vi "Donnees fichier distant.vi"() -> (0 "Données":string[](array[string]), 1 "données présentes":bool)   [LabVIEW 2022 SP3]
uses:
  Variables globales/Variable glob Keller.vi
  Variables globales/Variable glob Leybold.vi
  Variables globales/Variable glob Edwards.vi
  Variables globales/Variable glob Th.vi
  Variables globales/Variable glob Pt.vi
  Variables globales/Variables glob EUROTHERM.vi
  Variables globales/Variable globale compteurs.vi
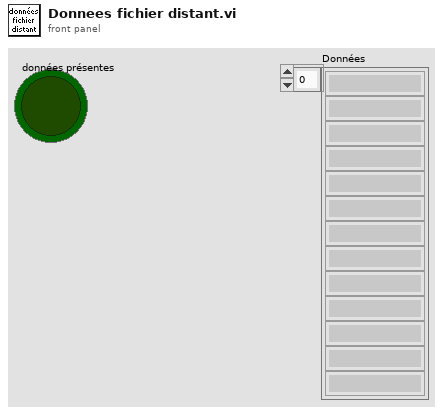
[diagram p1: front panel]
types:
  T1 = cluster{"Nom tache Pt":refnum<k21>, "Noms des Pt":string[], "Nb Pt":i16, "Selection Pt":bool[], "Nom Pt selectionnees":string[]}[]
  T2 = cluster{"Nom tache Th":refnum<k21>, "Noms des Th":string[], "Nb Th":i16, "Selection Th":bool[], "Nom Th selectionnes":string[]}[]
  T3 = cluster{"Nom tache compteurs":refnum<k21>, "Noms des compteurs":string[], "Selection":bool[], "Init compteurs":dbl[], "Noms compteurs selectionnes":string[]}
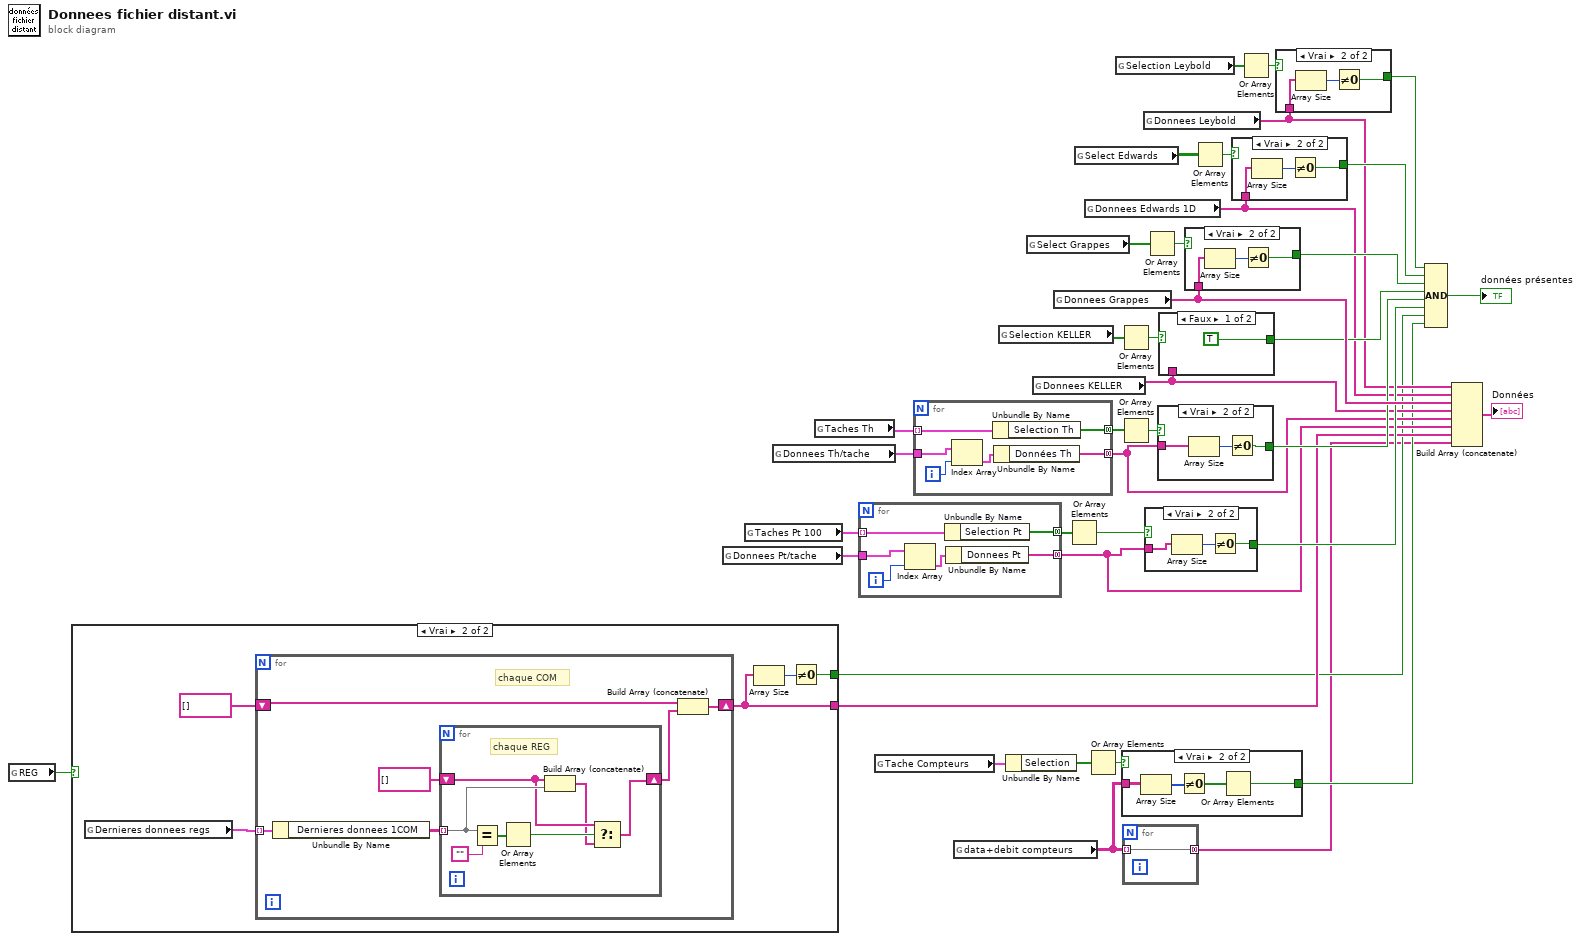
[diagram p0: block diagram]
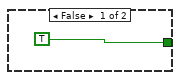
[diagram p2: hidden frame]
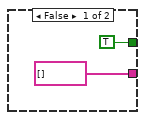
[diagram p3: hidden frame]
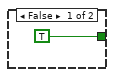
[diagram p4: hidden frame]
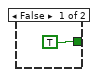
[diagram p5: hidden frame]
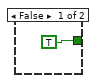
[diagram p6: hidden frame]
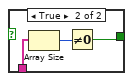
[diagram p7: hidden frame]
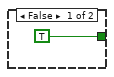
[diagram p8: hidden frame]
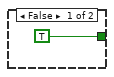
[diagram p9: hidden frame]
diagram:
  n1 = global read "Variables glob EUROTHERM.vi" "REG"() -> (w9:bool)
  n2 = case shown="Vrai" w9 {
    tunnel: [string[] [] w43] -> w8
    tunnel: [TRUE w42] -> w7
    frame False {
    }
    frame True {
      n3 = global read "Variables glob EUROTHERM.vi" "Dernieres donnees regs"() -> (w45:cluster{"Dernieres donnees 1COM":string[][]}[])
      n4 = for {
        tunnel: w45 -> [w48] mode=indexing
        shift-right: [w49] -> w43
        shift-left: string[] [] -> [w50]
        # "chaque COM"
        n5 = Unbundle By Name(w48) -> ("Dernieres donnees 1COM"=w47:string[][])
        n6 = for {
          tunnel: w47 -> [w59] mode=indexing
          shift-right: [w53] -> w51
          shift-left: string[] [] -> [w55]
          # "chaque REG"
          n7 = Equal?(x=w59, y="") -> (x = y?=w57:bool[])
          n8 = Or Array Elements(Boolean array=w57) -> (logical OR=w56:bool)
          n9 = Build Array (concatenate)(w55, w59) -> (w54:string[])
          n10 = Select(t=w55, s=w56, f=w54) -> (s? t:f=w53:string[])
        }
        n11 = Build Array (concatenate)(w50, w51) -> (w49:string[])
      }
      n12 = Array Size(array=w43) -> (size(s)=w44:i32)
      n13 = Not Equal To 0?(x=w44) -> (x != 0?=w42:bool)
    }
  }
  n14 = global read "Variable glob Pt.vi" "Donnees Pt/tache"() -> (w11:cluster{"Donnees Pt":string[]}[])
  n15 = global read "Variable glob Pt.vi" "Taches Pt 100"() -> (w17:T1)
  n16 = global read "Variable glob Th.vi" "Donnees Th/tache"() -> (w10:cluster{"Données Th":string[]}[])
  n17 = global read "Variable glob Th.vi" "Taches Th"() -> (w14:T2)
  n18 = for {
    tunnel: w17 -> [w64] mode=indexing
    tunnel: [w65] -> w16 mode=concatenating
    tunnel: [w63] -> w12 mode=concatenating
    tunnel: w11 -> [w61]
    i -> [w62]
    n19 = Index Array(array=w61, index=w62) -> (element=w60:cluster{"Donnees Pt":string[]})
    n20 = Unbundle By Name(w64) -> ("Selection Pt"=w65:bool[])
    n21 = Unbundle By Name(w60) -> ("Donnees Pt"=w63:string[])
  }
  n22 = global read "Variable globale compteurs.vi" "Tache Compteurs"() -> (w4:T3)
  n23 = for {
    tunnel: w14 -> [w71] mode=indexing
    tunnel: [w70] -> w15 mode=concatenating
    tunnel: [w69] -> w13 mode=concatenating
    tunnel: w10 -> [w68]
    i -> [w67]
    n24 = Index Array(array=w68, index=w67) -> (element=w66:cluster{"Données Th":string[]})
    n25 = Unbundle By Name(w71) -> ("Selection Th"=w70:bool[])
    n26 = Unbundle By Name(w66) -> ("Données Th"=w69:string[])
  }
  n27 = global read "Variable globale compteurs.vi" "data+debit compteurs"() -> (w6:string[][])
  n28 = global read "Variable glob Keller.vi" "Selection KELLER"() -> (w21:bool[])
  n29 = Unbundle By Name(w4) -> ("Selection"=w5:bool[])
  n30 = global read "Variable glob Edwards.vi" "Select Grappes"() -> (w37:bool[])
  n31 = global read "Variable glob Keller.vi" "Donnees KELLER"() -> (w28:string[])
  n32 = global read "Variable glob Edwards.vi" "Donnees Grappes"() -> (w38:string[])
  n33 = Or Array Elements(Boolean array=w16) -> (logical OR=w32:bool)
  n34 = global read "Variable glob Edwards.vi" "Select Edwards"() -> (w20:bool[][])
  n35 = global read "Variable glob Edwards.vi" "Donnees Edwards 1D"() -> (w25:string[])
  n36 = Or Array Elements(Boolean array=w5) -> (logical OR=w3:bool)
  n37 = global read "Variable glob Leybold.vi" "Selection Leybold"() -> (w18:bool[])
  n38 = Or Array Elements(Boolean array=w21) -> (logical OR=w27:bool)
  n39 = Or Array Elements(Boolean array=w15) -> (logical OR=w30:bool)
  n40 = case shown="Vrai" w3 {
    tunnel: w6 -> [_ w76]
    tunnel: [TRUE w73] -> w2
    frame False {
    }
    frame True {
      n41 = Array Size(array=w76) -> (size(s)=w75:i32[])
      n42 = Not Equal To 0?(x=w75) -> (x != 0?=w74:bool[])
      n43 = Or Array Elements(Boolean array=w74) -> (logical OR=w73:bool)
    }
  }
  n44 = for {
    tunnel: w6 -> [w77] mode=indexing
    tunnel: [w77] -> w1 mode=concatenating
  }
  n45 = global read "Variable glob Leybold.vi" "Donnees Leybold"() -> (w19:string[])
  n46 = case shown="Vrai" w32 {
    tunnel: [TRUE w80] -> w33
    tunnel: w12 -> [_ w79]
    frame False {
    }
    frame True {
      n47 = Array Size(array=w79) -> (size(s)=w81:i32)
      n48 = Not Equal To 0?(x=w81) -> (x != 0?=w80:bool)
    }
  }
  n49 = Or Array Elements(Boolean array=w37) -> (logical OR=w36:bool)
  n50 = case shown="Vrai" w30 {
    tunnel: [TRUE w84] -> w31
    tunnel: w13 -> [_ w83]
    frame False {
    }
    frame True {
      n51 = Array Size(array=w83) -> (size(s)=w85:i32)
      n52 = Not Equal To 0?(x=w85) -> (x != 0?=w84:bool)
    }
  }
  n53 = case shown="Faux" w27 {
    tunnel: w28 -> [_ w89]
    tunnel: [TRUE w87] -> w29
    frame False {
    }
    frame True {
      n54 = Array Size(array=w89) -> (size(s)=w88:i32)
      n55 = Not Equal To 0?(x=w88) -> (x != 0?=w87:bool)
    }
  }
  n56 = case shown="Vrai" w36 {
    tunnel: w38 -> [_ w93]
    tunnel: [TRUE w91] -> w39
    frame False {
    }
    frame True {
      n57 = Array Size(array=w93) -> (size(s)=w92:i32)
      n58 = Not Equal To 0?(x=w92) -> (x != 0?=w91:bool)
    }
  }
  n59 = Or Array Elements(Boolean array=w20) -> (logical OR=w24:bool)
  n60 = case shown="Vrai" w24 {
    tunnel: w25 -> [_ w97]
    tunnel: [TRUE w95] -> w26
    frame False {
    }
    frame True {
      n61 = Array Size(array=w97) -> (size(s)=w96:i32)
      n62 = Not Equal To 0?(x=w96) -> (x != 0?=w95:bool)
    }
  }
  n63 = Or Array Elements(Boolean array=w18) -> (logical OR=w22:bool)
  n64 = case shown="Vrai" w22 {
    tunnel: w19 -> [_ w101]
    tunnel: [TRUE w99] -> w23
    frame False {
    }
    frame True {
      n65 = Array Size(array=w101) -> (size(s)=w100:i32)
      n66 = Not Equal To 0?(x=w100) -> (x != 0?=w99:bool)
    }
  }
  n67 = Compound Arithmetic op=AND(w23, w26, w39, w29, w31, w33, w7, w2) -> (→"données présentes":bool)
  n68 = Build Array (concatenate)(w19, w25, w38, w28, w13, w12, w8, w1) -> (→"Données":string[])
